vi "Update Enum Getter.vi"(7 "RPC Message Name":string, 8 "error in (no error)":errorcluster, 10 "Message Getter in":refnum<vi>, 11 "RPC Messages Folder (ProjectItem) in":refnum<vi>) -> (0 "error out":errorcluster, 2 "Message Getter out":refnum<vi>, 3 "RPC Messages Folder (ProjectItem) out":refnum<vi>)   [LabVIEW 2019, in "gRPC Template Creation Utility.lvlib"]
uses:
  gRPC Template Creation Utility.lvlib
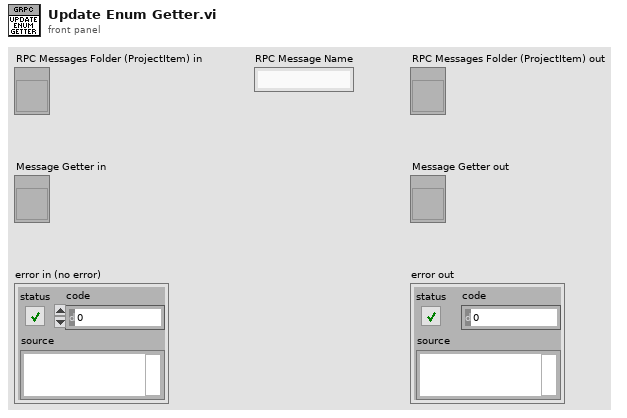
[diagram p1: front panel]
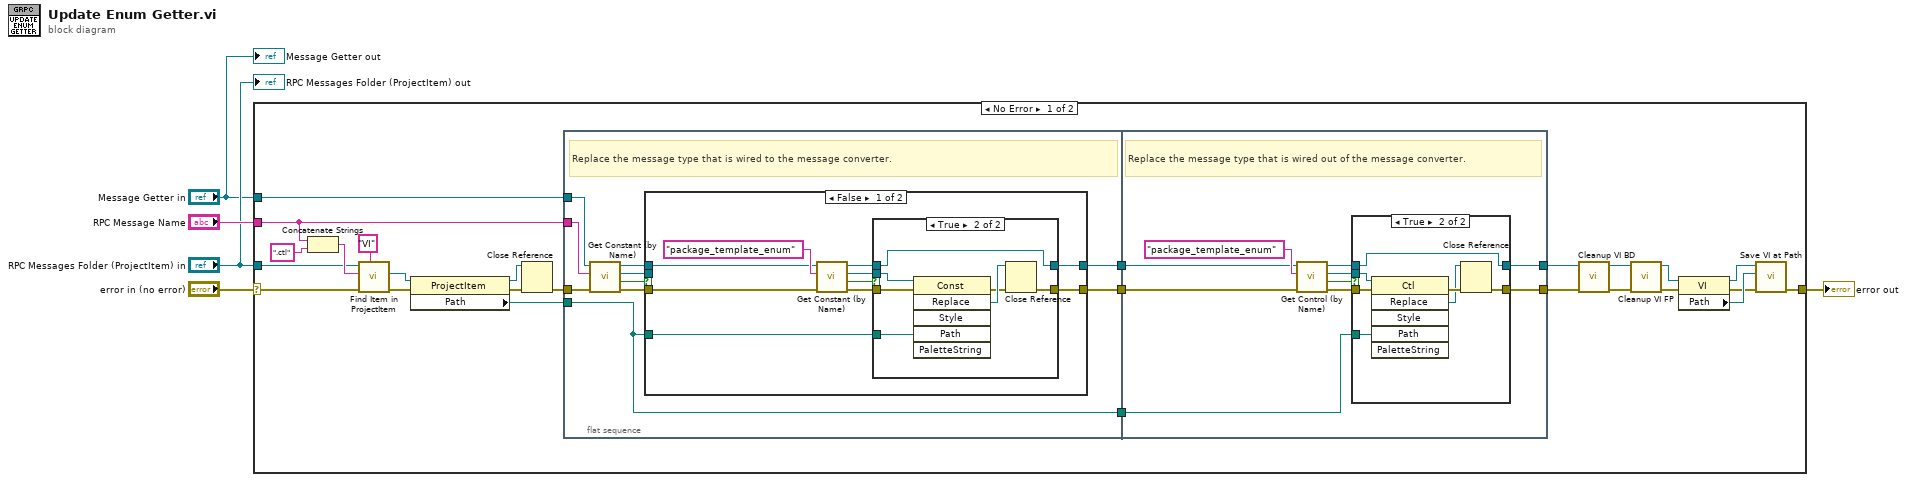
[diagram p0: block diagram]
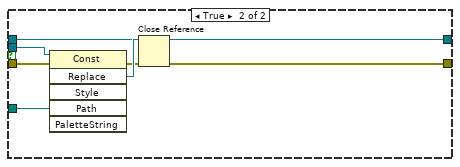
[diagram p3: hidden frame]
diagram:
  n1 = case shown="No Error" "error in (no error)" {
    selector: "error in (no error)" -> [w21 w87]
    tunnel: [w19 w87] -> w5
    tunnel: "RPC Message Name" -> [w22 _]
    tunnel: "RPC Messages Folder (ProjectItem) in" -> [w20 _]
    tunnel: "Message Getter in" -> [w17 _]
    frame No Error {
      n2 = Concatenate Strings(w22, ".ctl" ("string")) -> (w25:string)
      n3 = call "Find Item in ProjectItem.vi"("Item Type"="VI", "error in (no error)"=w21, "Name"=w25, "ProjectItem in"=w20) -> ("error out"=w29:errorcluster, "Item Refnum out"=w28:refnum<vi>)  [unwired: 4 in, 2 out]
      n4 = property class="ProjectItem"(reference=w28, error in=w29) -> (reference out=w30:refnum<vi>, error out=w31:errorcluster, "Path"=w23:path)
      n5 = Close Reference(reference=w30, error in (no error)=w31) -> (error out=w18:errorcluster)
      n6 = flat-sequence {
        tunnel: w23 -> [w32]
        tunnel: w18 -> [w40]
        tunnel: w22 -> [w39]
        tunnel: [w41] -> w24
        tunnel: w17 -> [w34]
        tunnel: [w33] -> w13
        tunnel: [w32] -> w12
        tunnel: w24 -> [w73]
        tunnel: w13 -> [w72]
        tunnel: w12 -> [w71]
        tunnel: [w68] -> w7
        tunnel: [w70] -> w9
        frame #0 {
          # "Replace the message type that is wired to the message converter."
          n7 = call "Get Constant (by Name).vi"("error in (no error)"=w40, "Constant Label"=w39, "Owner VI in"=w34) -> ("error out"=w38:errorcluster, "Found ?"=w37:bool, "Const ref out"=w36:refnum<vi>, "Owner VI out"=w35:refnum<vi>)  [unwired: 5 in]
          n8 = case shown="False" w37 {
            tunnel: [w51 w62] -> w41
            tunnel: w32 -> [w50 w63]
            tunnel: w38 -> [w45 w67]
            tunnel: w35 -> [w44 w61]
            tunnel: w36 -> [_ w66]
            tunnel: [w42 w61] -> w33
            frame False {
              n9 = call "Get Constant (by Name).vi"("error in (no error)"=w45, "Constant Label"="package_template_enum" ("name/order"), "Owner VI in"=w44) -> ("error out"=w47:errorcluster, "Found ?"=w46:bool, "Const ref out"=w49:refnum<vi>, "Owner VI out"=w43:refnum<vi>)  [unwired: 5 in]
              n10 = case shown="True" w46 {
                tunnel: [w53 w60] -> w51
                tunnel: w50 -> [_ w59]
                tunnel: w49 -> [_ w56]
                tunnel: w47 -> [w53 w55]
                tunnel: w43 -> [w52 w54]
                tunnel: [w52 w54] -> w42
                frame False {
                }
                frame True {
                  n11 = invoke class="Const" method="Replace"(reference=w56, error in=w55, "Path"=w59) -> (error out=w57:errorcluster, "Replace"=w58:refnum<vi>)  [unwired: 3 in, 4 out]
                  n12 = Close Reference(reference=w58, error in (no error)=w57) -> (error out=w60:errorcluster)
                }
              }
            }
            frame True {
              n13 = invoke class="Const" method="Replace"(reference=w66, error in=w67, "Path"=w63) -> (error out=w64:errorcluster, "Replace"=w65:refnum<vi>)  [unwired: 3 in, 4 out]
              n14 = Close Reference(reference=w65, error in (no error)=w64) -> (error out=w62:errorcluster)
            }
          }
        }
        frame #1 {
          # "Replace the message type that is wired out of the message converter."
          n15 = call "Get Control (by Name).vi"("error in (no error)"=w73, "Control Label"="package_template_enum" ("name/order"), "Owner VI in"=w72) -> ("error out"=w77:errorcluster, "Found ?"=w76:bool, "Control Refnum"=w75:refnum<vi>, "Owner VI out"=w69:refnum<vi>)  [unwired: 5 in]
          n16 = case shown="True" w76 {
            tunnel: [w79 w86] -> w70
            tunnel: w71 -> [_ w83]
            tunnel: w75 -> [_ w82]
            tunnel: w77 -> [w79 w81]
            tunnel: w69 -> [w78 w80]
            tunnel: [w78 w80] -> w68
            frame False {
            }
            frame True {
              n17 = invoke class="Ctl" method="Replace"(reference=w82, error in=w81, "Path"=w83) -> (error out=w85:errorcluster, "Replace"=w84:refnum<vi>)  [unwired: 3 in, 4 out]
              n18 = Close Reference(reference=w84, error in (no error)=w85) -> (error out=w86:errorcluster)
            }
          }
        }
      }
      n19 = call "Cleanup VI BD.vi"("error in (no error)"=w9, "VI in"=w7) -> ("error out"=w11:errorcluster, "VI out"=w10:refnum<vi>)  [unwired: 8 in]
      n20 = call "Cleanup VI FP.vi"("error in"=w11, "vi in"=w10) -> ("error out"=w8:errorcluster, "vi out"=w6:refnum<vi>)  [unwired: 8 in]
      n21 = property class="VI"(reference=w6, error in=w8) -> (reference out=w15:refnum<vi>, error out=w14:errorcluster, "Path"=w16:path)
      n22 = call "Save VI at Path.vi"("error in (no error)"=w14, "Path"=w16, "VI in"=w15) -> ("error out"=w19:errorcluster)  [unwired: 6 in, 2 out]
    }
    frame Error {
    }
  }
  "error out" <- w5
  "RPC Messages Folder (ProjectItem) out" <- "RPC Messages Folder (ProjectItem) in"
  "Message Getter out" <- "Message Getter in"
